vi "Hardware XML Write (Ballard-1533).vi"(6 "ballard_bus hw map":T1, 8 "error in":errorcluster, 10 "configuration":T3[](array[typedef]), 11 "xml ref in":refnum<k24>) -> (0 "error out":errorcluster, 3 "xml ref out":refnum<k24>)   [LabVIEW 2020]
uses:
  C:/Users/Administrator/Desktop/GIT/Ballard-MIL-STD-1553-Custom-Device/Source/System Explorer/SubVIs/Parse XML Ballard/1.2/BTIXML_SerDes.dll
  Ballard-MIL-STD-1553-Custom-Device/Source/System Explorer/SubVIs/Parse XML Ballard/1.2/BTIXML_SerDes.dll
  _controls/ballard1553_cluster.ctl
  _controls/aim1553_messages.ctl
  _controls/1553_Parameters_key.ctl
  _controls/1553_Parameters.ctl
  _controls/1553_minorFrames.ctl
  _controls/ballard1553_hw_map.ctl
  _controls/ballard1553_RT_list.ctl
  Libraries/Ballard_1553_Hardware_ni/_typedefs/core_sequentialLog_type.ctl
  Libraries/Ballard_1553_Hardware_ni/_typedefs/MessageCommand_BCRT_type.ctl
  Libraries/Ballard_1553_Hardware_ni/_typedefs/MessageCommand_RTRT_type.ctl
  Libraries/Ballard_1553_Hardware_ni/_typedefs/RemoteTerminal_type.ctl
  Libraries/Ballard_1553_Hardware_ni/_typedefs/subAddress_type.ctl
  Libraries/Ballard_1553_Hardware_ni/Ballard_1553_Hardware_ni.lvlib
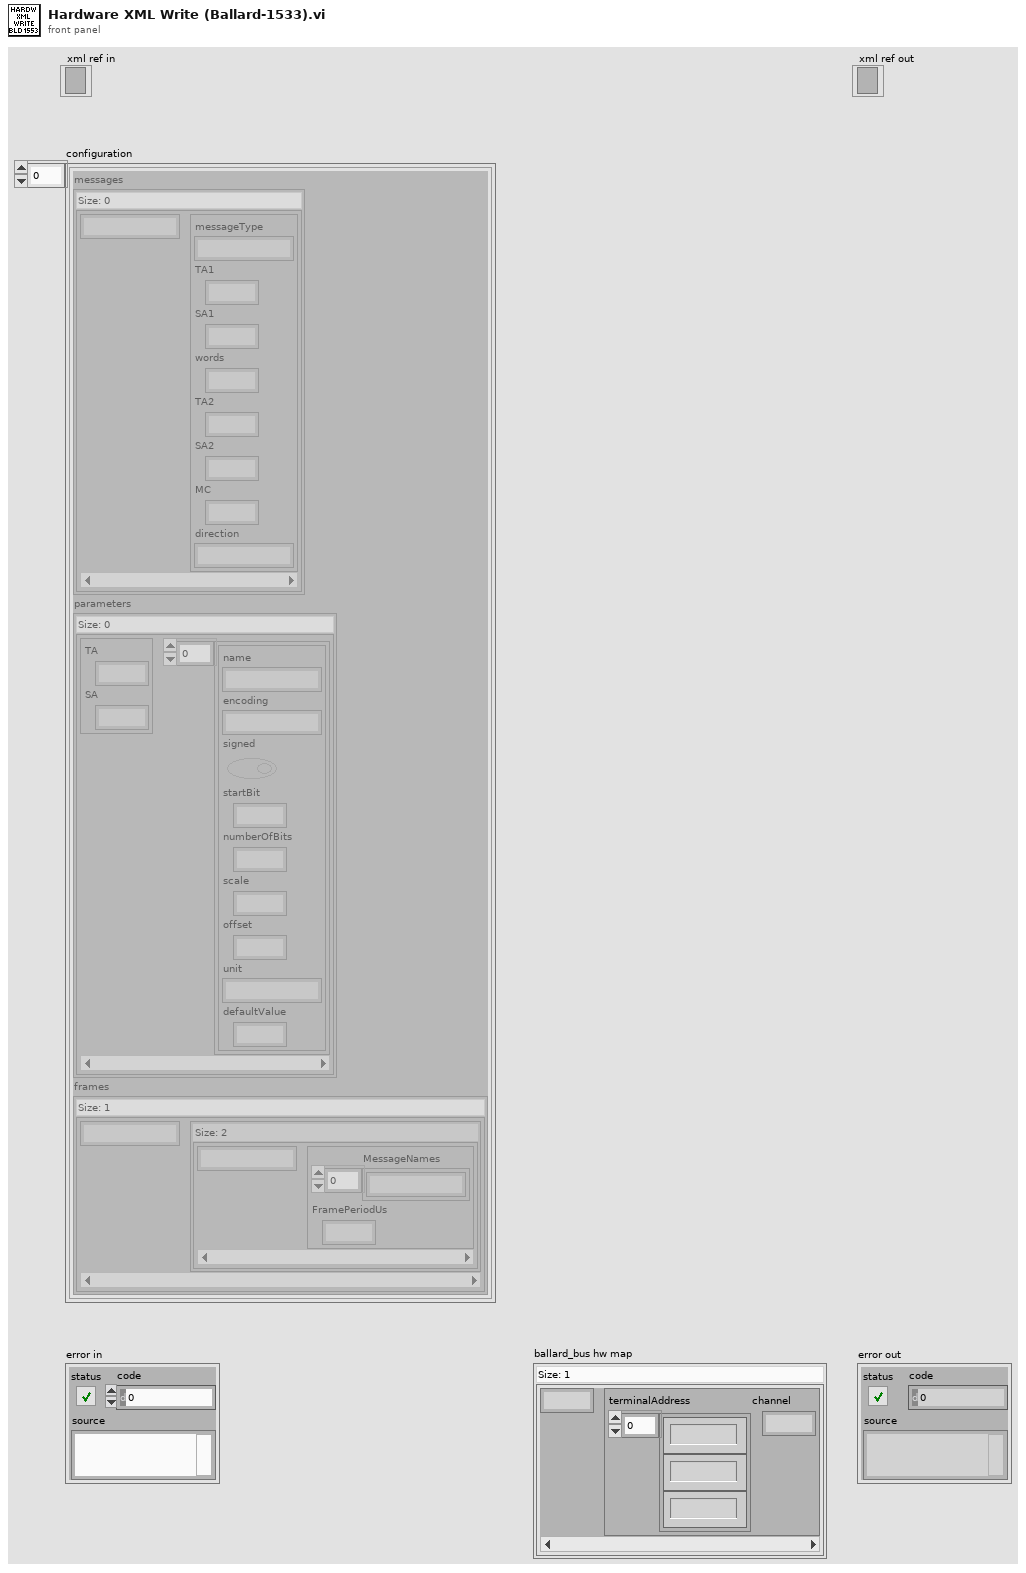
[diagram p1: front panel]
types:
  T1 = typedef "ballard1553_hw_map.ctl" = map{i32, T2}
  T2 = typedef "ballard1553_RT_list.ctl" = cluster{"terminalAddress":i32[], "channel":i32}
  T3 = typedef "ballard1553_cluster.ctl" = cluster{"messages":map{string, T4}, "parameters":map{T5, T6[]}, "frames":map{string, map{string, T7}}}
  T4 = typedef "aim1553_messages.ctl" = cluster{"messageType":string, "TA1":i32, "SA1":i32, "words":i32, "TA2":i32, "SA2":i32, "MC":i32, "direction":string}
  T5 = typedef "1553_Parameters_key.ctl" = cluster{"TA":i32, "SA":i32}
  T6 = typedef "1553_Parameters.ctl" = cluster{"name":string, "encoding":string, "signed":bool, "startBit":i32, "numberOfBits":i32, "scale":dbl, "offset":dbl, "unit":string, "defaultValue":dbl}
  T7 = typedef "1553_minorFrames.ctl" = cluster{"MessageNames":string[], "FramePeriodUs":i32}
  T8 = typedef "Ballard_1553_Hardware_ni.lvlib/core_sequentialLog_type.ctl" = cluster{"perChannelStreaming (T)":bool, "useDMA (T)":bool}
  T9 = typedef "Ballard_1553_Hardware_ni.lvlib/MessageCommand_BCRT_type.ctl" = cluster{"taVal1":i8, "saVal1":i8, "wordCount1":i8}
  T10 = typedef "Ballard_1553_Hardware_ni.lvlib/MessageCommand_RTRT_type.ctl" = cluster{"taVal1":i8, "saVal1":i8, "wordCount1":i8, "taVal2":i8, "saVal2":i8, "wordCount2":i8}
  T11 = typedef "Ballard_1553_Hardware_ni.lvlib/RemoteTerminal_type.ctl" = cluster{"rtAddress":i8, "rtMode":i32, "initialSwd":u8[], "noBuild":bool, "autoBusy":bool, "dynamicBC":bool, "clearSwdImmediate":bool, "busEnable":i32, "dataWipe":i32, "syncMode":i32, "responseMode":i32, "responseTime":dbl}
  T12 = typedef "Ballard_1553_Hardware_ni.lvlib/subAddress_type.ctl" = cluster{"enable":bool, "dataWipe":i32, "allowErrorInjection":bool, "eventLog":bool, "syncOutput":bool, "monitor":bool, "timeOrHitCount":i32, "elapseMinOrMax":i32, "wrap":bool}
  T13 = typedef "Ballard_1553_Hardware_ni.lvlib/schedItem1553_type.ctl" = cluster{"type":T14, "messageIDRef":i32, "singleShot (F)":bool, "skip (F)":bool, "gapTime":dbl}
  T14 = typedef "Ballard_1553_Hardware_ni.lvlib/frame_entry_type.ctl" = enum16{"Message", "Gap", "Pulse", "Log", "Pause", "Restart", "Halt"}
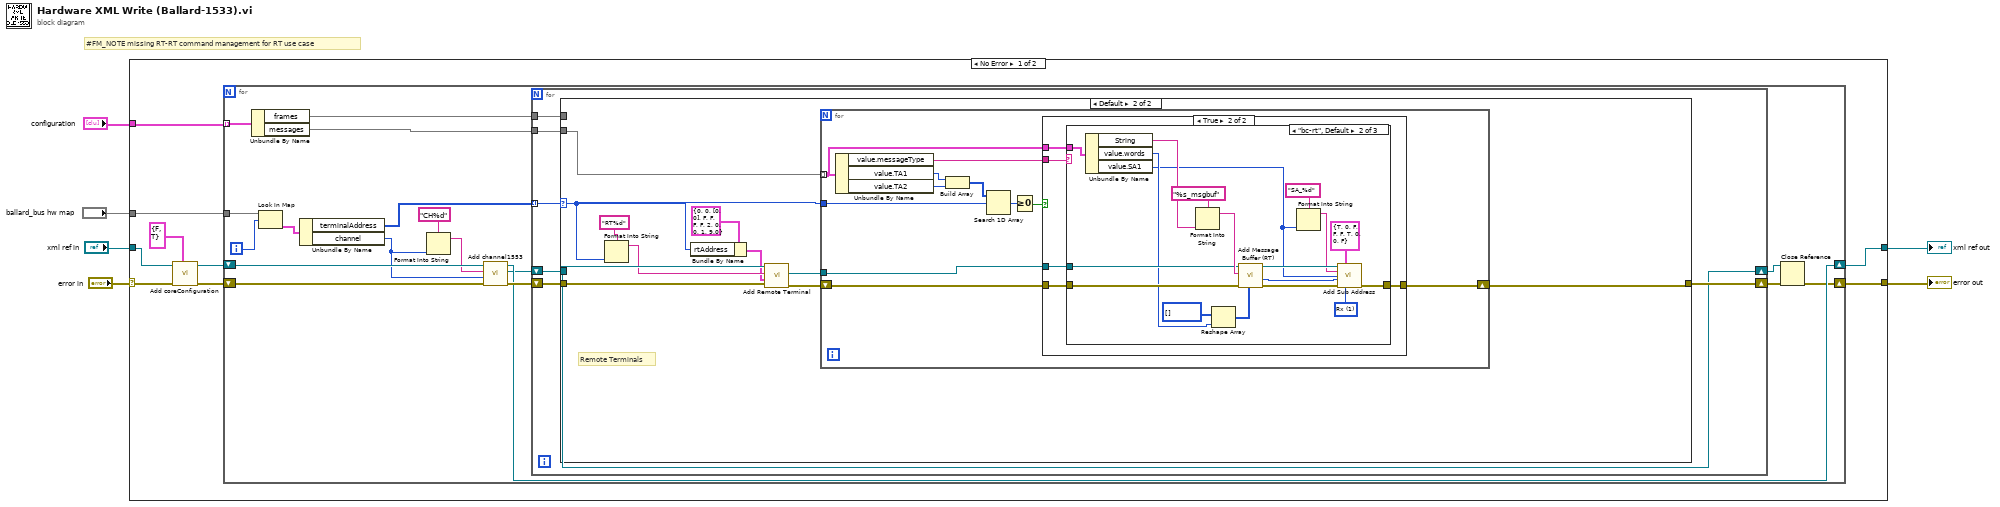
[diagram p0: block diagram]
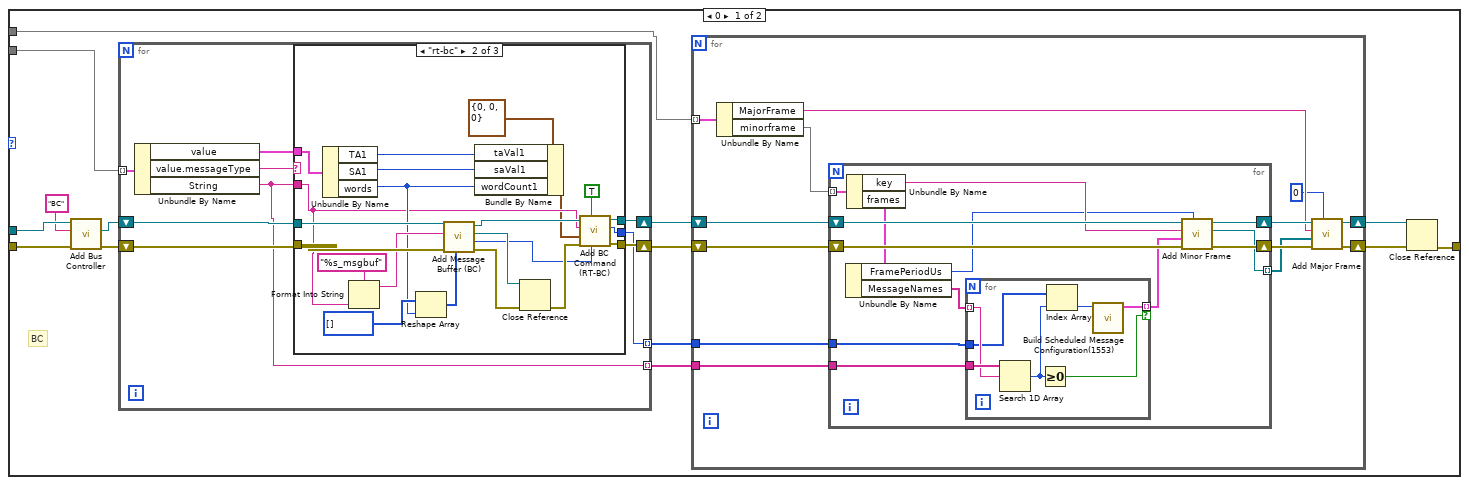
[diagram p2: hidden frame]
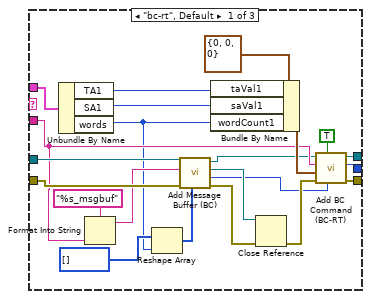
[diagram p3: hidden frame]
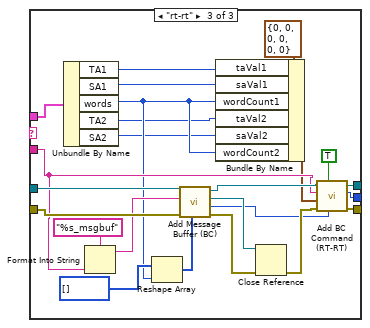
[diagram p4: hidden frame]
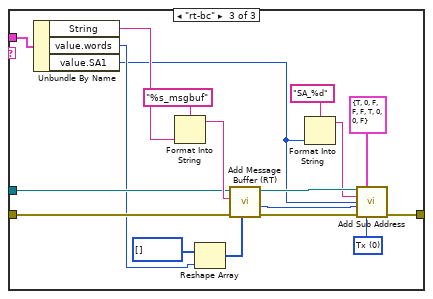
[diagram p7: hidden frame]
diagram:
  # "#FM_NOTE missing RT-RT command management for RT use case"
  n1 = case shown="No Error" "error in" {
    selector: "error in" -> [w15 w229]
    tunnel: "xml ref in" -> [w14 w230]
    tunnel: [w11 w230] -> w4
    tunnel: [w10 w229] -> w3
    tunnel: "configuration" -> [w9 _]
    tunnel: "ballard_bus hw map" -> [w8 _]
    frame No Error {
      n2 = call "Add coreConfiguration.vi"("core sequentialLog configuration (default)"=T8 {"perChannelStreaming (T)"=FALSE, "useDMA (T)"=TRUE}, "error in"=w15, "xml ref in"=w14) -> ("error out"=w12:errorcluster, "xml ref out"=w13:refnum<k24>)  [unwired: 6 in, 1 out]
      n3 = for {
        shift-right: [w17] -> w10
        shift-left: w12 -> [w32]
        shift-right: [w23] -> w11
        shift-left: w13 -> [w33]
        tunnel: w9 -> [w30] mode=indexing
        tunnel: w8 -> [w31]
        i -> [w29]
        n4 = Unbundle By Name(w30) -> ("frames"=w19:map{string, map{string, T7}}, "messages"=w20:map{string, T4})
        n5 = Look In Map(map=w31, key=w29) -> (value=w28:T2)  [unwired: 1 in, 1 out]
        n6 = Unbundle By Name(w28) -> ("terminalAddress"=w21:i32[], "channel"=w27:i32)
        n7 = Format Into String(format string="CH%d", w27) -> (resulting string=w25:string)  [unwired: 2 in, 1 out]
        n8 = call "Add channel1553.vi"("error in"=w32, "hardwareChannel (-1)"=w27, "name"=w25, "xml ref in"=w33) -> ("error out"=w24:errorcluster, "new channel1553 out"=w22:refnum<k24>, "xml ref out"=w23:refnum<k24>)  [unwired: 5 in]
        n9 = for {
          tunnel: w21 -> [w38] mode=indexing
          tunnel: w20 -> [w37]
          tunnel: w19 -> [w36]
          shift-right: [w34] -> w18
          shift-left: w22 -> [w34]
          shift-right: [w35] -> w16
          shift-left: w24 -> [w39]
          n10 = case shown="Default" w38 {
            selector: w38 -> [_ w164]
            tunnel: w39 -> [w53 w174]
            tunnel: w34 -> [w52 w173]
            tunnel: w37 -> [w50 w170]
            tunnel: w36 -> [w42 _]
            tunnel: [w45 w168] -> w35
            frame 0 {
              # "BC"
              n11 = call "Add Bus Controller.vi"("error in"=w53, "name"="BC", "1553channel ref in"=w52) -> ("error out"=w49:errorcluster, "new busController"=w48:refnum<k24>)  [unwired: 6 in, 1 out]
              n12 = for {
                tunnel: w50 -> [w95] mode=indexing
                shift-right: [w92] -> w47
                shift-left: w49 -> [w89]
                shift-right: [w91] -> w43
                shift-left: w48 -> [w88]
                tunnel: [w87] -> w40 mode=indexing
                tunnel: [w90] -> w41 mode=indexing
                n13 = Unbundle By Name(w95) -> ("value"=w93:T4, "value.messageType"=w94:string, "String"=w87:string)
                n14 = case shown="\"rt-bc\"" w94 {
                  tunnel: w89 -> [w106 w132 w156]
                  tunnel: w93 -> [w116 w139 w163]
                  tunnel: w88 -> [w107 w133 w157]
                  tunnel: [w117 w120 w147] -> w92
                  tunnel: w87 -> [w103 w125 w150]
                  tunnel: [w111 w122 w145] -> w91
                  tunnel: [w110 w121 w146] -> w90
                  frame "bc-rt", Default {
                    n15 = Unbundle By Name(w116) -> ("TA1"=w113:i32, "SA1"=w112:i32, "words"=w100:i32)
                    n16 = Format Into String(format string="%s_msgbuf", w103) -> (resulting string=w102:string)  [unwired: 2 in, 1 out]
                    n17 = Reshape Array(u16[] [] ("MessageData (0x0000)"), w100) -> (w99:u16[])
                    n18 = call "Add Message Buffer (BC).vi"("MessageData (0x0000)"=w99, "error in"=w106, "name"=w102, "Bus Controllerl in"=w107) -> ("error out"=w109:errorcluster, "ID out"=w97:i32, "new messageBuffer"=w108:refnum<k24>, "Bus Controller out"=w98:refnum<k24>)  [unwired: 4 in]
                    n19 = Bundle By Name(cluster=T9 {"taVal1"=0, "saVal1"=0, "wordCount1"=0} ("Message Command Configuration"), "taVal1"=w113, "saVal1"=w112, "wordCount1"=w100) -> (w114:T9)
                    n20 = Close Reference(reference=w108, error in (no error)=w109) -> (error out=w105:errorcluster)
                    n21 = call "Add BC Command (BC-RT).vi"("messageBufferIDRef(-1)"=w97, "monitor (F)"=TRUE, "error in"=w105, "Message Command Configuration"=w114, "name"=w103, "BusController in"=w98) -> ("error out"=w117:errorcluster, "Message Command ID out"=w110:i32, "BusController out"=w111:refnum<k24>)  [unwired: 3 in]
                  }
                  frame "rt-bc" {
                    n22 = Unbundle By Name(w139) -> ("TA1"=w137:i32, "SA1"=w136:i32, "words"=w128:i32)
                    n23 = Format Into String(format string="%s_msgbuf", w125) -> (resulting string=w130:string)  [unwired: 2 in, 1 out]
                    n24 = Reshape Array(u16[] [] ("MessageData (0x0000)"), w128) -> (w127:u16[])
                    n25 = call "Add Message Buffer (BC).vi"("MessageData (0x0000)"=w127, "error in"=w132, "name"=w130, "Bus Controllerl in"=w133) -> ("error out"=w135:errorcluster, "ID out"=w119:i32, "new messageBuffer"=w134:refnum<k24>, "Bus Controller out"=w126:refnum<k24>)  [unwired: 4 in]
                    n26 = Bundle By Name(cluster=T9 {"taVal1"=0, "saVal1"=0, "wordCount1"=0} ("Message Command Configuration"), "taVal1"=w137, "saVal1"=w136, "wordCount1"=w128) -> (w124:T9)
                    n27 = Close Reference(reference=w134, error in (no error)=w135) -> (error out=w123:errorcluster)
                    n28 = call "Add BC Command (RT-BC).vi"("messageBufferIDRef(-1)"=w119, "monitor(F)"=TRUE, "error in"=w123, "Message Command Configuration"=w124, "name"=w125, "BusController in"=w126) -> ("error out"=w120:errorcluster, "Message Command ID out"=w121:i32, "BusController out"=w122:refnum<k24>)  [unwired: 3 in]
                  }
                  frame "rt-rt" {
                    n29 = Unbundle By Name(w163) -> ("TA1"=w161:i32, "SA1"=w160:i32, "words"=w144:i32, "TA2"=w143:i32, "SA2"=w142:i32)
                    n30 = Format Into String(format string="%s_msgbuf", w150) -> (resulting string=w154:string)  [unwired: 2 in, 1 out]
                    n31 = Reshape Array(u16[] [] ("MessageData (0x0000)"), w144) -> (w152:u16[])
                    n32 = call "Add Message Buffer (BC).vi"("MessageData (0x0000)"=w152, "error in"=w156, "name"=w154, "Bus Controllerl in"=w157) -> ("error out"=w159:errorcluster, "ID out"=w141:i32, "new messageBuffer"=w158:refnum<k24>, "Bus Controller out"=w151:refnum<k24>)  [unwired: 4 in]
                    n33 = Bundle By Name(cluster=T10 {"taVal1"=0, "saVal1"=0, "wordCount1"=0, "taVal2"=0, "saVal2"=0, "wordCount2"=0} ("Message Command Configuration"), "taVal1"=w161, "saVal1"=w160, "wordCount1"=w144, "taVal2"=w143, "saVal2"=w142, "wordCount2"=w144) -> (w148:T10)
                    n34 = Close Reference(reference=w158, error in (no error)=w159) -> (error out=w149:errorcluster)
                    n35 = call "Add BC Command (RT-RT).vi"("messageBufferIDRef(-1)"=w141, "monitor(F)"=TRUE, "error in"=w149, "Message Command Configuration"=w148, "name"=w150, "BusController in"=w151) -> ("error out"=w147:errorcluster, "Message Command ID out"=w146:i32, "BusController out"=w145:refnum<k24>)  [unwired: 3 in]
                  }
                }
              }
              n36 = for {
                shift-right: [w64] -> w46
                shift-left: w47 -> [w66]
                shift-right: [w63] -> w44
                shift-left: w43 -> [w62]
                tunnel: w42 -> [w60] mode=indexing
                tunnel: w41 -> [w55]
                tunnel: w40 -> [w56]
                n37 = Unbundle By Name(w60) -> ("MajorFrame"=w59:string, "minorframe"=w58:map{string, T7})
                n38 = for {
                  shift-right: [w78] -> w65
                  shift-left: w66 -> [w79]
                  shift-right: [w76] -> w61
                  shift-left: w62 -> [w77]
                  tunnel: w58 -> [w75] mode=indexing
                  tunnel: [w69] -> w57 mode=indexing
                  tunnel: w56 -> [w68]
                  tunnel: w55 -> [w67]
                  n39 = Unbundle By Name(w75) -> ("key"=w74:string, "frames"=w73:T7)
                  n40 = Unbundle By Name(w73) -> ("FramePeriodUs"=w72:i32, "MessageNames"=w71:string[])
                  n41 = for {
                    tunnel: w71 -> [w84] mode=indexing
                    tunnel: [w86] -> w70 mode=indexing if=w83
                    tunnel: w68 -> [w85]
                    tunnel: w67 -> [w82]
                    n42 = Search 1D Array(1D array=w85, element=w84) -> (index of element=w81:i32)  [unwired: 1 in]
                    n43 = Greater Or Equal To 0?(x=w81) -> (x >= 0?=w83:bool)
                    n44 = Index Array(array=w82, index=w81) -> (element=w80:i32)
                    n45 = call "Build Scheduled Message Configuration(1553).vi"("messageIDRef"=w80) -> ("1553 Scheduled Message Configuration out"=w86:T13)  [unwired: 10 in]
                  }
                  n46 = call "Add Minor Frame.vi"("frameTime uS (200)"=w72, "error in"=w79, "Scheduled Message Config in"=w70, "name"=w74, "BusController in"=w77) -> ("error out"=w78:errorcluster, "new Minor Frame"=w69:refnum<k24>, "BusController out"=w76:refnum<k24>)  [unwired: 4 in]
                }
                n47 = call "Add Major Frame.vi"("loopCount (0: continous)"=0, "error in"=w65, "Minor Frames"=w57, "name"=w59, "BusController in"=w61) -> ("error out"=w64:errorcluster, "BusController out"=w63:refnum<k24>)  [unwired: 5 in]
              }
              n48 = Close Reference(reference=w44, error in (no error)=w46) -> (error out=w45:errorcluster)
            }
            frame Default {
              # "Remote Terminals"
              n49 = Format Into String(format string="RT%d", w164) -> (resulting string=w171:string)  [unwired: 2 in, 1 out]
              n50 = Bundle By Name(cluster=T11 {"rtAddress"=0, "rtMode"=0, "initialSwd"=[0, 0], "noBuild"=FALSE, "autoBusy"=FALSE, "dynamicBC"=FALSE, "clearSwdImmediate"=FALSE, "busEnable"=2, "dataWipe"=0, "syncMode"=0, "responseMode"=1, "responseTime"=9.0} ("Remote Terminal Config"), "rtAddress"=w164) -> (w165:T11)
              n51 = call "Add Remote Terminal.vi"("error in"=w174, "Remote Terminal Config"=w165, "name"=w171, "1553channel ref in"=w173) -> ("error out"=w169:errorcluster, "new remoteTerminal"=w167:refnum<k24>)  [unwired: 5 in, 1 out]
              n52 = for {
                tunnel: w170 -> [w179] mode=indexing
                shift-right: [w175] -> w168
                shift-left: w169 -> [w184]
                tunnel: w167 -> [w185]
                tunnel: w164 -> [w180]
                n53 = Unbundle By Name(w179) -> ("value.messageType"=w176:string, "value.TA1"=w183:i32, "value.TA2"=w182:i32)
                n54 = Build Array(w183, w182) -> (w181:i32[])
                n55 = Search 1D Array(1D array=w181, element=w180) -> (index of element=w177:i32)  [unwired: 1 in]
                n56 = Greater Or Equal To 0?(x=w177) -> (x >= 0?=w178:bool)
                n57 = case shown="True" w178 {
                  tunnel: w185 -> [_ w191]
                  tunnel: w184 -> [w186 w190]
                  tunnel: w179 -> [_ w189]
                  tunnel: w176 -> [_ w188]
                  tunnel: [w186 w187] -> w175
                  frame False {
                  }
                  frame True {
                    n58 = case shown="\"bc-rt\", Default" w188 {
                      tunnel: w191 -> [_ w208 w226]
                      tunnel: w190 -> [w192 w207 w225]
                      tunnel: w189 -> [_ w205 w223]
                      tunnel: [w192 w195 w213] -> w187
                      frame "False" {
                      }
                      frame "bc-rt", Default {
                        w194 = 1 items=["Tx", "Rx"] ("direction (Tx)")
                        n59 = Unbundle By Name(w205) -> ("String"=w204:string, "value.words"=w203:i32, "value.SA1"=w199:i32)
                        n60 = Format Into String(format string="%s_msgbuf", w204) -> (resulting string=w209:string)  [unwired: 2 in, 1 out]
                        n61 = Reshape Array(u16[] [] ("MessageData (0x0000)"), w203) -> (w202:u16[])
                        n62 = call "Add Message Buffer (RT).vi"("MessageData (0x0000)"=w202, "error in"=w207, "name"=w209, "Remote Terminal in"=w208) -> ("error out"=w196:errorcluster, "ID out"=w197:i32, "Remote Terminal out"=w201:refnum<k24>)  [unwired: 4 in, 1 out]
                        n63 = Format Into String(format string="SA_%d", w199) -> (resulting string=w198:string)  [unwired: 2 in, 1 out]
                        n64 = call "Add Sub Address.vi"("Remote Terminal in"=w201, "SubAddress Config"=T12 {"enable"=TRUE, "dataWipe"=0, "allowErrorInjection"=FALSE, "eventLog"=FALSE, "syncOutput"=FALSE, "monitor"=TRUE, "timeOrHitCount"=0, "elapseMinOrMax"=0, "wrap"=FALSE}, "name"=w198, "subAddress"=w199, "messageBufferIDRef (-1)"=w197, "error in"=w196, "direction (Tx)"=w194) -> ("error out"=w195:errorcluster)  [unwired: 5 in, 3 out]
                      }
                      frame "rt-bc" {
                        w212 = 0 items=["Tx", "Rx"] ("direction (Tx)")
                        n65 = Unbundle By Name(w223) -> ("String"=w222:string, "value.words"=w221:i32, "value.SA1"=w217:i32)
                        n66 = Format Into String(format string="%s_msgbuf", w222) -> (resulting string=w227:string)  [unwired: 2 in, 1 out]
                        n67 = Reshape Array(u16[] [] ("MessageData (0x0000)"), w221) -> (w220:u16[])
                        n68 = call "Add Message Buffer (RT).vi"("MessageData (0x0000)"=w220, "error in"=w225, "name"=w227, "Remote Terminal in"=w226) -> ("error out"=w214:errorcluster, "ID out"=w215:i32, "Remote Terminal out"=w219:refnum<k24>)  [unwired: 4 in, 1 out]
                        n69 = Format Into String(format string="SA_%d", w217) -> (resulting string=w216:string)  [unwired: 2 in, 1 out]
                        n70 = call "Add Sub Address.vi"("Remote Terminal in"=w219, "SubAddress Config"=T12 {"enable"=TRUE, "dataWipe"=0, "allowErrorInjection"=FALSE, "eventLog"=FALSE, "syncOutput"=FALSE, "monitor"=TRUE, "timeOrHitCount"=0, "elapseMinOrMax"=0, "wrap"=FALSE}, "name"=w216, "subAddress"=w217, "messageBufferIDRef (-1)"=w215, "error in"=w214, "direction (Tx)"=w212) -> ("error out"=w213:errorcluster)  [unwired: 5 in, 3 out]
                      }
                    }
                  }
                }
              }
            }
          }
        }
        n71 = Close Reference(reference=w18, error in (no error)=w16) -> (error out=w17:errorcluster)
      }
    }
    frame Error {
    }
  }
  "xml ref out" <- w4
  "error out" <- w3
